vi "filter possible timestamps.vi"(5 "SecondsSinceStart":dbl, 7 "engine start":timestamp, 8 "seconds at start":dbl, 9 "step time":timestamp, 10 "numerics":T2[](array[typedef]), 11 "strings":T4(array[cluster])) -> (0 "possible timestamp numeric matches":T3(c390), 1 "possible timestamp string matches":T1(c390), 2 "remaining numerics":T2[](array[typedef]), 3 "remaining strings":T4(array[cluster]))   [LabVIEW 2020, in "nominal teststand model sequence support.lvlib"]
doc: "takes all result strings and numerics and attempts to remove items that have certain keys in the name (_ts, _time, _timestamp) at the end of the name.\n\nFor strings, it will parse as a labview representation of a teststand timestamp (teststand doesn't support labview's timestamp type, so it stores it as a string which...sigh).\n\nFor numerics it will attempt to guess which epoch the timestamp is part of (teststand engine 1970, teststand start time (time - start time relative to 1970), or standard labview time 1904)."
uses:
  nominal teststand model sequence support.lvlib
  nominal numeric result collection.ctl
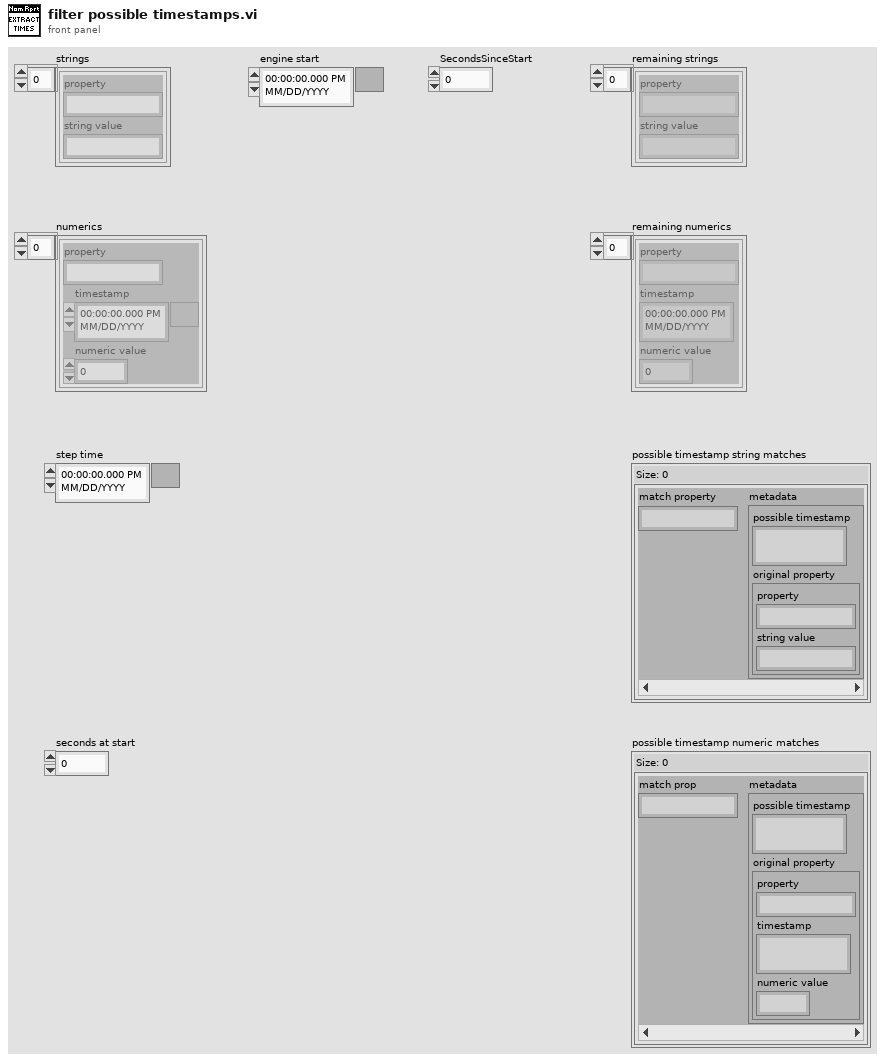
[diagram p1: front panel]
types:
  T1 = map{string, cluster{"possible timestamp":timestamp, "original property":cluster{"property":string, "string value":string}}}
  T2 = typedef "nominal teststand model sequence support.lvlib/nominal numeric result collection.ctl" = cluster{"property":string, "timestamp":timestamp, "numeric value":dbl}
  T3 = map{string, cluster{"possible timestamp":timestamp, "original property":T2}}
  T4 = cluster{"property":string, "string value":string}[]
  T5 = cluster{"property":string, "Cluster":cluster{"property":string, "string value":string}}
  T6 = map{string, cluster{timestamp, "original property":T2}}
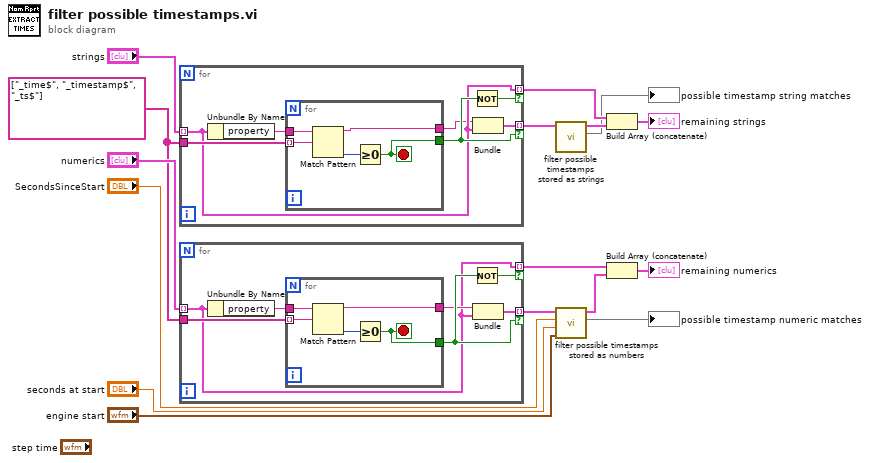
[diagram p0: block diagram]
diagram:
  w14 = string[] ["_time$", "_timestamp$", "_ts$"]
  n1 = for {
    tunnel: "strings" -> [w19] mode=indexing
    tunnel: [w19] -> w11 mode=indexing if=w22
    tunnel: [w17] -> w12 mode=indexing if=w23
    tunnel: w14 -> [w20]
    n2 = Unbundle By Name(w19) -> ("property"=w21:string)
    n3 = for {
      tunnel: [w25] -> w23
      tunnel: w21 -> [w27]
      tunnel: w20 -> [w26] mode=indexing
      tunnel: [w24] -> w18
      stop <- w25 stop-if-true
      n4 = Match Pattern(string=w27, regular expression=w26) -> (before substring=w24:string, offset past match=w28:i32)  [unwired: 1 in, 2 out]
      n5 = Greater Or Equal To 0?(x=w28) -> (x >= 0?=w25:bool)
    }
    n6 = Not(x=w23) -> (.not. x?=w22:bool)
    n7 = Bundle("property"=w18, "Cluster"=w19) -> (w17:T5)  [unwired: 1 in]
  }
  n8 = for {
    tunnel: "numerics" -> [w30] mode=indexing
    tunnel: [w30] -> w13 mode=indexing if=w34
    tunnel: [w29] -> w3 mode=indexing if=w35
    tunnel: w14 -> [w32]
    n9 = Unbundle By Name(w30) -> ("property"=w33:string)
    n10 = for {
      tunnel: [w37] -> w35
      tunnel: w33 -> [w39]
      tunnel: w32 -> [w38] mode=indexing
      tunnel: [w36] -> w31
      stop <- w37 stop-if-true
      n11 = Match Pattern(string=w39, regular expression=w38) -> (before substring=w36:string, offset past match=w40:i32)  [unwired: 1 in, 2 out]
      n12 = Greater Or Equal To 0?(x=w40) -> (x >= 0?=w37:bool)
    }
    n13 = Not(x=w35) -> (.not. x?=w34:bool)
    n14 = Bundle("property"=w31, "Cluster"=w30) -> (w29:cluster{"property":string, "Cluster":T2})  [unwired: 1 in]
  }
  n15 = call "filter possible timestamps stored as strings.vi"("possible timestamps"=w12) -> ("property-to-match -> timestamp and original prop"=→"possible timestamp string matches":T1, "remaining properties"=w9:T4)  [unwired: 9 in]
  n16 = call "filter possible timestamps stored as numbers.vi"("engine start"="engine start", "seconds at start"="seconds at start", "SecondsSinceStart"="SecondsSinceStart", "Array in"=w3) -> ("property-to-match -> timestamp + original property"=→"possible timestamp numeric matches":T6, "unmatched numerics"=w7:T2[])  [unwired: 6 in]
  n17 = Build Array (concatenate)(w11, w9) -> (→"remaining strings":T4)
  n18 = Build Array (concatenate)(w13, w7) -> (→"remaining numerics":T2[])
